vi "RemoteVI Point On Popup.vi"(0 "windows":T1(array[cluster]), 5 "x":i32, 7 "y":i32) -> (4 "on popup?":bool, 6 "index":i32=-1)   [LabVIEW 2020, in "RemoteVI.lvlib"]
doc: "TRUE when the screen point (x, y) lies inside any of windows (logical rectangles, right and bottom exclusive); index is the first such window - windows are listed top-most first, so that is the one on top - or -1 when none. Pure."
uses:
  RemoteVI.lvlib
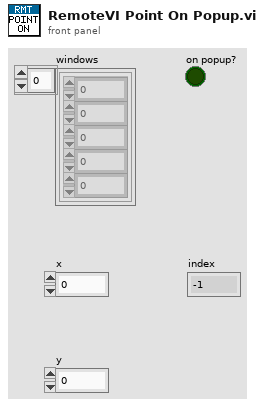
[diagram p1: front panel]
types:
  T1 = cluster{"hwnd":u64, "x":i32, "y":i32, "w":i32, "h":i32}[]
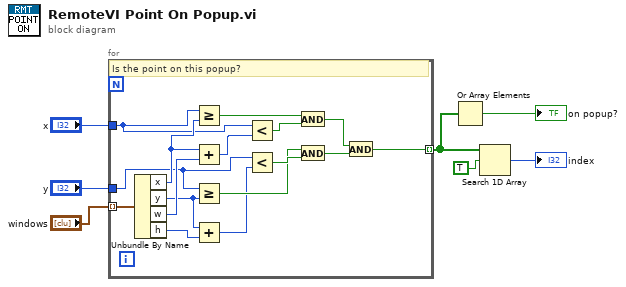
[diagram p0: block diagram]
diagram:
  n1 = for {
    tunnel: "windows" -> [w8] mode=indexing
    tunnel: "x" -> [w9]
    tunnel: "y" -> [w10]
    tunnel: [w23] -> w4 mode=indexing
    # "Is the point on this popup?"
    n2 = Unbundle By Name(w8) -> ("x"=w11:i32, "y"=w12:i32, "w"=w13:i32, "h"=w14:i32)
    n3 = Greater Or Equal?(x=w9, y=w11) -> (x >= y?=w17:bool)
    n4 = Add(x=w11, y=w13) -> (x+y=w15:i32)
    n5 = Greater Or Equal?(x=w10, y=w12) -> (x >= y?=w19:bool)
    n6 = Add(x=w12, y=w14) -> (x+y=w16:i32)
    n7 = Less?(x=w9, y=w15) -> (x < y?=w18:bool)
    n8 = Less?(x=w10, y=w16) -> (x < y?=w20:bool)
    n9 = And(x=w17, y=w18) -> (x .and. y?=w21:bool)
    n10 = And(x=w19, y=w20) -> (x .and. y?=w22:bool)
    n11 = And(x=w21, y=w22) -> (x .and. y?=w23:bool)
  }
  n12 = Or Array Elements(Boolean array=w4) -> (logical OR=→"on popup?":bool)
  n13 = Search 1D Array(1D array=w4, element=TRUE) -> (index of element=→"index":i32)  [unwired: 1 in]
